vi "Jay'sCameraSystemTest.vi"() -> (3 "Servo Command":T1)   [LabVIEW 2026]
uses:
  Typedefs/ServoCommand.ctl
  <vilib>/vision/Image Controls.llb/IMAQ Image.ctl
panel:
  in  "Min circularity":dbl=1.08
  in  "20mm Cube max area":dbl=140000.0
  in  "20mm Cube min area":dbl=110000.0
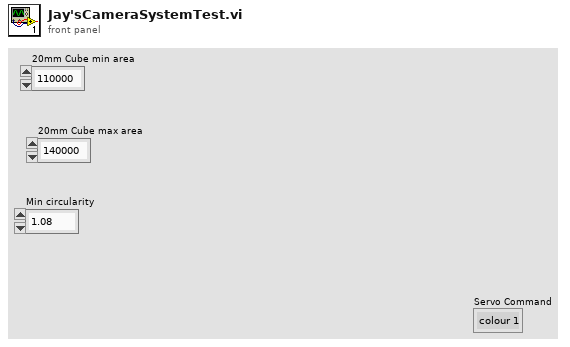
[diagram p1: front panel]
types:
  T1 = typedef "ServoCommand.ctl" = enum16{"colour 1", "Colour2", "Colour3", "Reject"}
  T2 = typedef "IMAQ Image.ctl" = refnum<image>
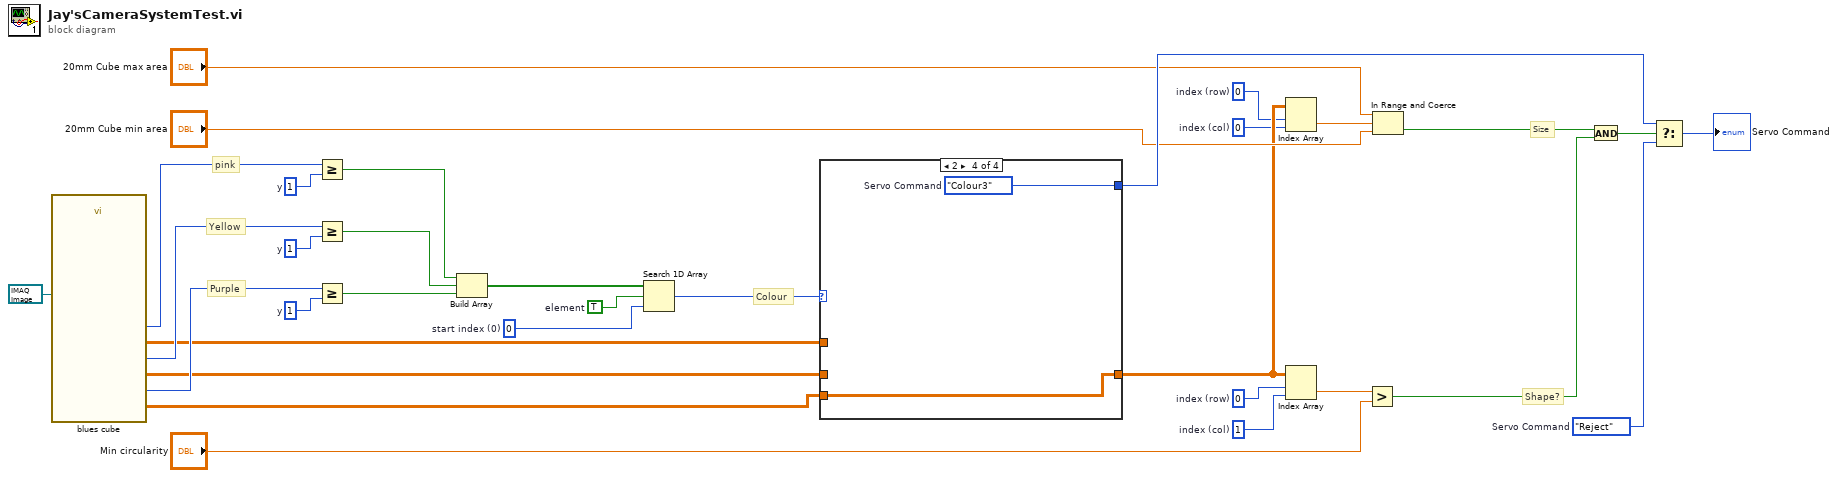
[diagram p0: block diagram]
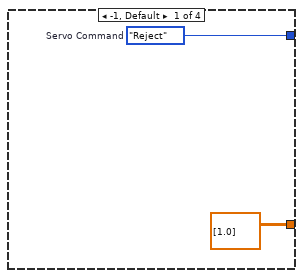
[diagram p2: hidden frame]
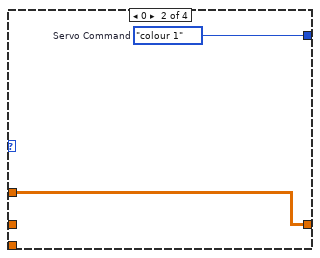
[diagram p3: hidden frame]
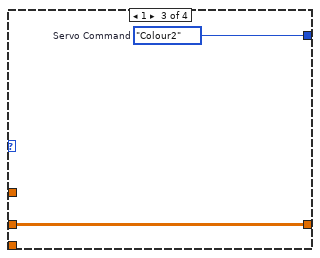
[diagram p4: hidden frame]
diagram:
  w12 = 1  # index (col)
  w13 = 0  # index (col)
  w17 = 0  # index (row)
  w15 = 0  # index (row)
  w19 = TRUE  # element
  w20 = 0  # start index (0)
  w26 = ServoCommand."Reject"  # Servo Command
  w31 = 1  # y
  w32 = 1  # y
  w33 = 1  # y
  # "Colour"
  # "Shape?"
  # "Size"
  # "Yellow"
  # "pink"
  # "Purple"
  n1 = call "blues cube"("Image In"=T2 refnum) -> ("Particle Measurements (Pixels) (Analyse pink object)"=w4:dbl[][], "Particle Measurements (Pixels) (Analyse yellow object)"=w3:dbl[][], "Particle Measurements (Pixels) (Analyse Purple object)"=w2:dbl[][], "Number of Particles (Analyse pink object)"=w7:i32, "Number of Particles (Analyse yellow object)"=w6:i32, "Number of Particles (Analyse Purple object)"=w5:i32)  [unwired: 19 in, 2 out]
  n2 = Greater Or Equal?(x=w7, y=w33) -> (x >= y?=w30:bool)
  n3 = Greater Or Equal?(x=w6, y=w32) -> (x >= y?=w29:bool)
  n4 = Greater Or Equal?(x=w5, y=w31) -> (x >= y?=w28:bool)
  n5 = Build Array "Build Array"(w30, w29, w28) -> (w21:bool[])
  n6 = Search 1D Array(1D array=w21, element=w19, start index (0)=w20) -> (index of element=w18:i32)
  n7 = case shown="2" w18 {
    tunnel: [w35 w37 w39 w41] -> w27
    tunnel: [dbl[][] [[1.0]] w36 w38 w40] -> w16
    tunnel: w4 -> [_ w36 _ _]
    tunnel: w3 -> [_ _ w38 _]
    tunnel: w2 -> [_ _ _ w40]
    frame -1, Default {
      w35 = ServoCommand."Reject"  # Servo Command
    }
    frame 0 {
      w37 = ServoCommand."colour 1"  # Servo Command
    }
    frame 1 {
      w39 = ServoCommand."Colour2"  # Servo Command
    }
    frame 2 {
      w41 = ServoCommand."Colour3"  # Servo Command
    }
  }
  n8 = Index Array "Index Array"(array=w16, index (row)=w15, index (col)=w13) -> (element=w14:dbl)
  n9 = Index Array "Index Array"(array=w16, index (row)=w17, index (col)=w12) -> (element=w10:dbl)
  n10 = Greater?(x=w10, y="Min circularity") -> (0:w8:bool)
  n11 = In Range and Coerce(upper limit="20mm Cube max area", x=w14, lower limit="20mm Cube min area") -> (In Range?=w22:bool)  [unwired: 1 out]
  n12 = And(x=w22, y=w8) -> (x .and. y?=w11:bool)
  n13 = Select(t=w27, s=w11, f=w26) -> (s? t:f=→"Servo Command":T1)
